vi "Get Server Type and Status.vi"(0 "All Interfaces Dict":variant, 2 "Specific Interface Dict in":variant, 3 "Listener Settings":T1, 5 "error in (no error)":errorcluster) -> (14 "Is \"All Interface\" Server":bool, 15 "Server Running":bool, 16 "Server URI":string, 19 "error out":errorcluster)   [LabVIEW 2016, in "WebSocket Actors.lvlib" / "WebSocket Server Manager.lvclass"]
uses:
  WebSocket Server Manager.lvclass
  WebSocket Server/typedefs/Listener Settings.ctl
  WebSocket Server/WebSocket Server.lvclass
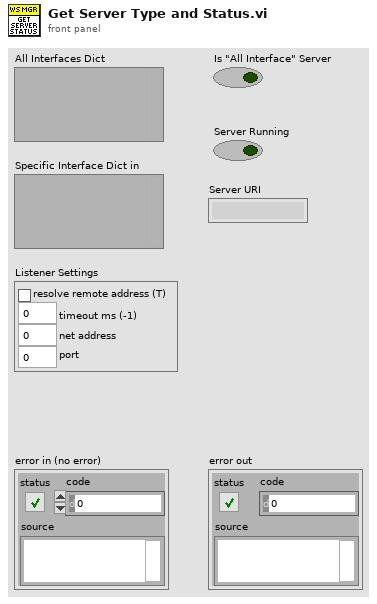
[diagram p1: front panel]
types:
  T1 = typedef "WebSocket Actors.lvlib/WebSocket Server.lvclass/Listener Settings.ctl" = cluster{"resolve remote address (T)":bool, "timeout ms (-1)":i32, "net address":u32, "port":u16}
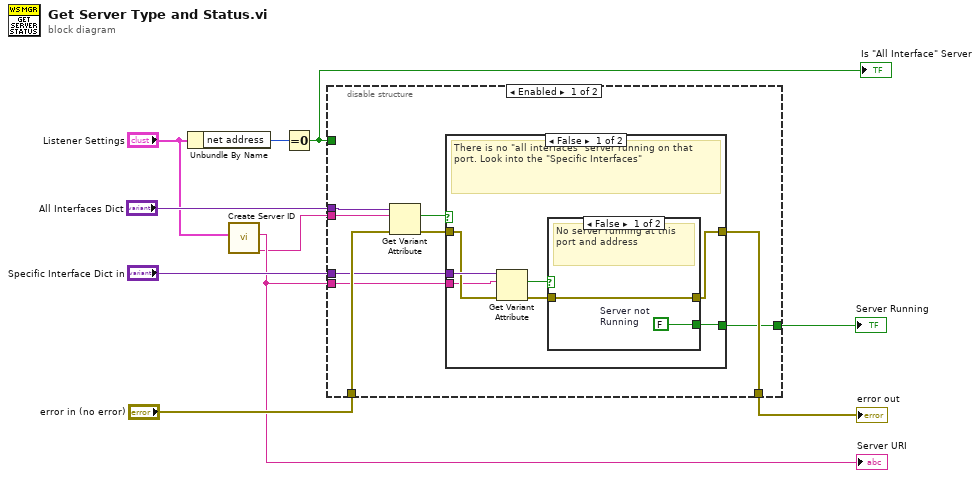
[diagram p0: block diagram]
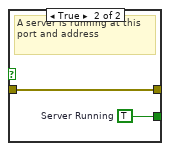
[diagram p2: hidden frame]
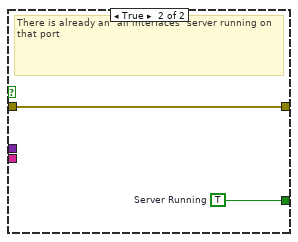
[diagram p3: hidden frame]
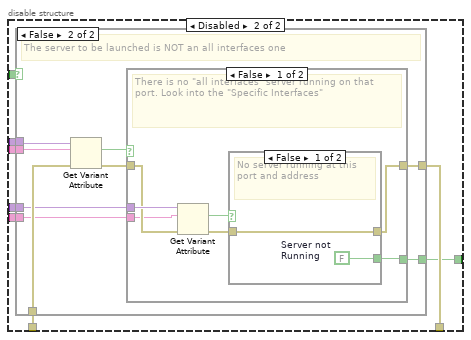
[diagram p4: hidden frame]
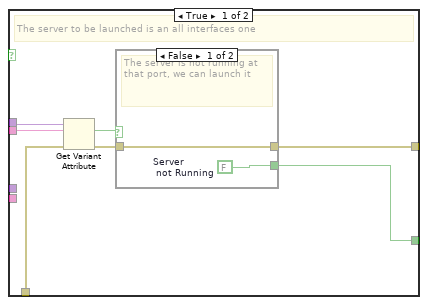
[diagram p5: hidden frame]
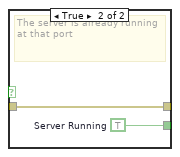
[diagram p6: hidden frame]
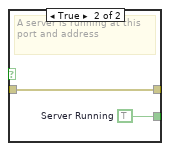
[diagram p7: hidden frame]
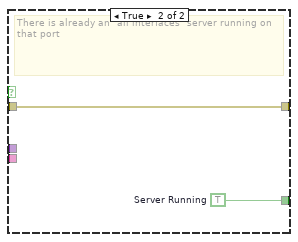
[diagram p8: hidden frame]
diagram:
  n1 = Unbundle By Name("Listener Settings") -> ("net address"=w4:u32)
  n2 = call "Create Server ID.vi"("Listener Settings"="Listener Settings") -> ("Port String"=w1:string, "Server URI"=w2:string)  [unwired: 7 in, 1 out]
  "Server URI" <- w2
  n3 = Equal To 0?(x=w4) -> (x = 0?=w9:bool)
  "Is \"All Interface\" Server" <- w9
  n4 = disable-structure shown="Enabled" {
    disable-tunnel: [w19 w40] -> w10
    disable-tunnel: w9 -> [_ w39]
    disable-tunnel: [w18 w38] -> w8
    disable-tunnel: "error in (no error)" -> [w17 w37]
    disable-tunnel: "All Interfaces Dict" -> [w16 w36]
    disable-tunnel: "Specific Interface Dict in" -> [w15 w35]
    disable-tunnel: w2 -> [w14 w34]
    disable-tunnel: w1 -> [w13 w33]
    frame Enabled {
      n5 = Get Variant Attribute(Variant=w16, name=w13, error in=w17) -> (found=w12:bool, error out=w11:errorcluster)  [unwired: 1 in, 2 out]
      n6 = case shown="False" w12 {
        tunnel: w11 -> [w25 w31]
        tunnel: [w20 w31] -> w19
        tunnel: [w21 w32] -> w18
        tunnel: w15 -> [w26 _]
        tunnel: w14 -> [w24 _]
        frame False {
          # "There is no \"all interfaces\" server running on that port. Look into the \"Specific Interfaces\""
          n7 = Get Variant Attribute(Variant=w26, name=w24, error in=w25) -> (found=w23:bool, error out=w22:errorcluster)  [unwired: 1 in, 2 out]
          n8 = case shown="False" w23 {
            tunnel: w22 -> [w27 w29]
            tunnel: [w28 w30] -> w21
            tunnel: [w27 w29] -> w20
            frame False {
              w28 = FALSE  # Server not  Running
              # "No server running at this port and address"
            }
            frame True {
              w30 = TRUE  # Server Running
              # "A server is running at this port and address"
            }
          }
        }
        frame True {
          w32 = TRUE  # Server Running
          # "There is already an \"all interfaces\" server running on that port"
        }
      }
    }
    frame Disabled {
      n9 = case shown="False" w39 {
        tunnel: w35 -> [_ w56]
        tunnel: w36 -> [w47 w60]
        tunnel: w33 -> [w45 w53]
        tunnel: w37 -> [w44 w58]
        tunnel: [w42 w54] -> w40
        tunnel: [w41 w55] -> w38
        tunnel: w34 -> [_ w52]
        frame True {
          # "The server to be launched is an all interfaces one"
          n10 = Get Variant Attribute(Variant=w47, name=w45, error in=w44) -> (found=w46:bool, error out=w43:errorcluster)  [unwired: 1 in, 2 out]
          n11 = case shown="False" w46 {
            tunnel: w43 -> [w49 w50]
            tunnel: [w49 w50] -> w42
            tunnel: [w48 w51] -> w41
            frame False {
              w48 = FALSE  # Server  not Running
              # "The server is not running at that port, we can launch it"
            }
            frame True {
              w51 = TRUE  # Server Running
              # "The server is already running at that port"
            }
          }
        }
        frame False {
          # "The server to be launched is NOT an all interfaces one"
          n12 = Get Variant Attribute(Variant=w60, name=w53, error in=w58) -> (found=w59:bool, error out=w57:errorcluster)  [unwired: 1 in, 2 out]
          n13 = case shown="False" w59 {
            tunnel: w57 -> [w66 w72]
            tunnel: [w61 w72] -> w54
            tunnel: [w62 w73] -> w55
            tunnel: w56 -> [w67 _]
            tunnel: w52 -> [w65 _]
            frame False {
              # "There is no \"all interfaces\" server running on that port. Look into the \"Specific Interfaces\""
              n14 = Get Variant Attribute(Variant=w67, name=w65, error in=w66) -> (found=w64:bool, error out=w63:errorcluster)  [unwired: 1 in, 2 out]
              n15 = case shown="False" w64 {
                tunnel: w63 -> [w68 w70]
                tunnel: [w69 w71] -> w62
                tunnel: [w68 w70] -> w61
                frame False {
                  w69 = FALSE  # Server not  Running
                  # "No server running at this port and address"
                }
                frame True {
                  w71 = TRUE  # Server Running
                  # "A server is running at this port and address"
                }
              }
            }
            frame True {
              w73 = TRUE  # Server Running
              # "There is already an \"all interfaces\" server running on that port"
            }
          }
        }
      }
    }
  }
  "error out" <- w10
  "Server Running" <- w8
